vi "Update RPC Template Accessor.vi"(8 "error in (no error)":errorcluster, 10 "Accessor Name":string, 11 "Server Library (Library Item) in":refnum<vi>) -> (0 "error out":errorcluster, 3 "Server Library (Library Item) out":refnum<vi>)   [LabVIEW 2019, in "gRPC Template Creation Utility.lvlib"]
uses:
  gRPC Template Creation Utility.lvlib
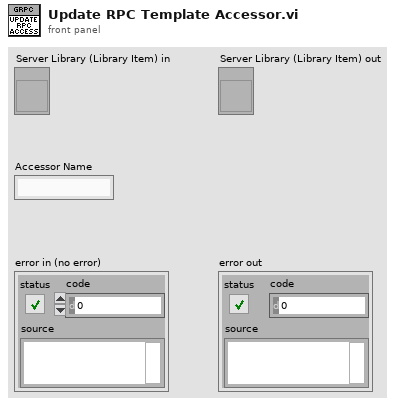
[diagram p1: front panel]
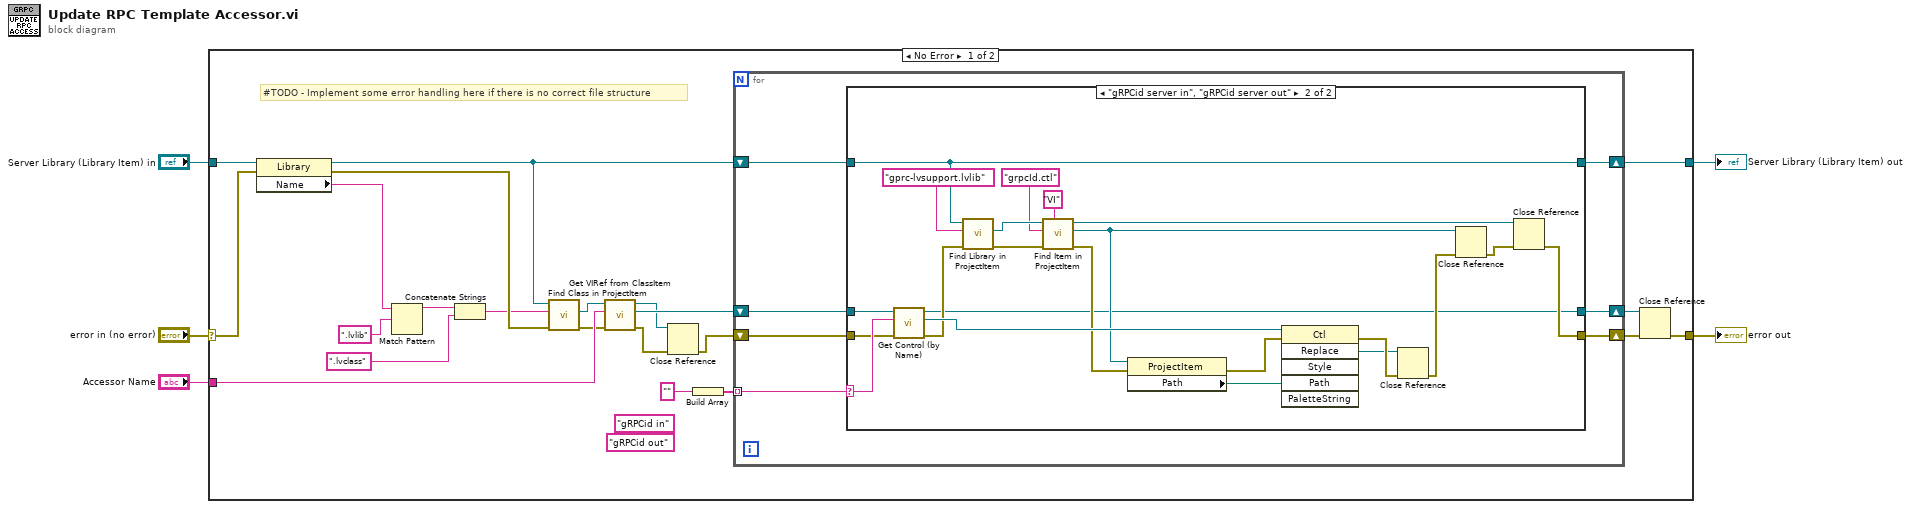
[diagram p0: block diagram]
diagram:
  n1 = case shown="No Error" "error in (no error)" {
    selector: "error in (no error)" -> [w12 w60]
    tunnel: [w27 w61] -> w5
    tunnel: "Server Library (Library Item) in" -> [w14 w61]
    tunnel: "Accessor Name" -> [w24 _]
    tunnel: [w21 w60] -> w2
    frame No Error {
      (unwired) "gRPCid out" ("Item Name")
      (unwired) "gRPCid in" ("Item Name")
      # "#TODO - Implement some error handling here if there is no correct file structure"
      n2 = property class="Library"(reference=w14, error in=w12) -> (reference out=w13:refnum<vi>, error out=w20:errorcluster, "Name"=w17:string)
      n3 = Match Pattern(string=w17, regular expression=".lvlib") -> (before substring=w18:string)  [unwired: 1 in, 3 out]
      n4 = Concatenate Strings(w18, ".lvclass" ("string")) -> (w19:string)
      n5 = call "Find Class in ProjectItem.vi"("error in (no error)"=w20, "Class Name"=w19, "ProjectItem in"=w13) -> ("error out"=w11:errorcluster, "LVClass out"=w9:refnum<vi>)  [unwired: 5 in, 2 out]
      n6 = call "Get VIRef from ClassItem.vi"("error in (no error)"=w11, "Item Name"=w24, "LVClassLibrary in"=w9) -> ("error out"=w10:errorcluster, "VIref out"=w25:refnum<vi>, "LVClassLibrary out"=w6:refnum<vi>)  [unwired: 5 in, 1 out]
      n7 = Close Reference(reference=w6, error in (no error)=w10) -> (error out=w8:errorcluster)
      n8 = Build Array("") -> (w26:string[])
      n9 = for {
        tunnel: w26 -> [w34] mode=indexing
        shift-right: [w32] -> w27
        shift-left: w13 -> [w33]
        shift-right: [w29] -> w23
        shift-left: w8 -> [w30]
        shift-right: [w28] -> w22
        shift-left: w25 -> [w31]
        n10 = case shown="\"gRPCid server in\", \"gRPCid server out\"" w34 {
          selector: w34 -> [_ w42]
          tunnel: w33 -> [w37 w43]
          tunnel: [w37 w43] -> w32
          tunnel: w31 -> [w36 w39]
          tunnel: w30 -> [w35 w41]
          tunnel: [w35 w40] -> w29
          tunnel: [w36 w38] -> w28
          frame "False", Default {
          }
          frame "gRPCid server in", "gRPCid server out" {
            n11 = call "Get Control (by Name).vi"("error in (no error)"=w41, "Control Label"=w42, "Owner VI in"=w39) -> ("error out"=w53:errorcluster, "Control Refnum"=w55:refnum<vi>, "Owner VI out"=w38:refnum<vi>)  [unwired: 5 in, 1 out]
            n12 = call "Find Library in ProjectItem.vi"("error in (no error)"=w53, "Library Name"="gprc-lvsupport.lvlib", "ProjectItem in"=w43) -> ("error out"=w52:errorcluster, "Library out"=w58:refnum<vi>)  [unwired: 5 in, 2 out]
            n13 = call "Find Item in ProjectItem.vi"("Item Type"="VI", "error in (no error)"=w52, "Name"="grpcId.ctl", "ProjectItem in"=w58) -> ("error out"=w51:errorcluster, "Item Refnum out"=w46:refnum<vi>, "ProjectItem out"=w44:refnum<vi>)  [unwired: 4 in, 1 out]
            n14 = property class="ProjectItem"(reference=w46, error in=w51) -> (error out=w48:errorcluster, "Path"=w54:path)  [unwired: 1 out]
            n15 = invoke class="Ctl" method="Replace"(reference=w55, error in=w48, "Path"=w54) -> (error out=w50:errorcluster, "Replace"=w49:refnum<vi>)  [unwired: 3 in, 4 out]
            n16 = Close Reference(reference=w49, error in (no error)=w50) -> (error out=w47:errorcluster)
            n17 = Close Reference(reference=w46, error in (no error)=w47) -> (error out=w45:errorcluster)
            n18 = Close Reference(reference=w44, error in (no error)=w45) -> (error out=w40:errorcluster)
          }
        }
      }
      n19 = Close Reference(reference=w22, error in (no error)=w23) -> (error out=w21:errorcluster)
    }
    frame Error {
    }
  }
  "Server Library (Library Item) out" <- w5
  "error out" <- w2
